vi "Status_Call.vi"(8 "error in (no error)":errorcluster, 9 "connection":T3={"host"="", "channel"=2, "cert path"=path "/home/lvuser/cansub_root_cert.crt"}, 10 "open in":bool, 11 "status client in":T2) -> (0 "error out":errorcluster, 1 "device status":T1, 2 "open out":bool, 3 "status client out":T2)   [LabVIEW 2021, in "CANsub_API.lvlib"]
doc: "Reads the device status with an HTTPS client that stays open between calls. Opens the client on the first call (about 80 ms for the TLS handshake). A later call takes about 1 ms. After an error, the client is closed, and the next call opens a new one."
uses:
  CANsub_API.lvlib
  common/CANsub_Common.lvlib
  <vilib>/httpClient/ClientHandle.ctl
  <vilib>/httpClient/LabVIEWHTTPClient.lvlib
  common/Typedefs/CANsub_connection.ctl
  common/Typedefs/CANsub_Device_Status.ctl
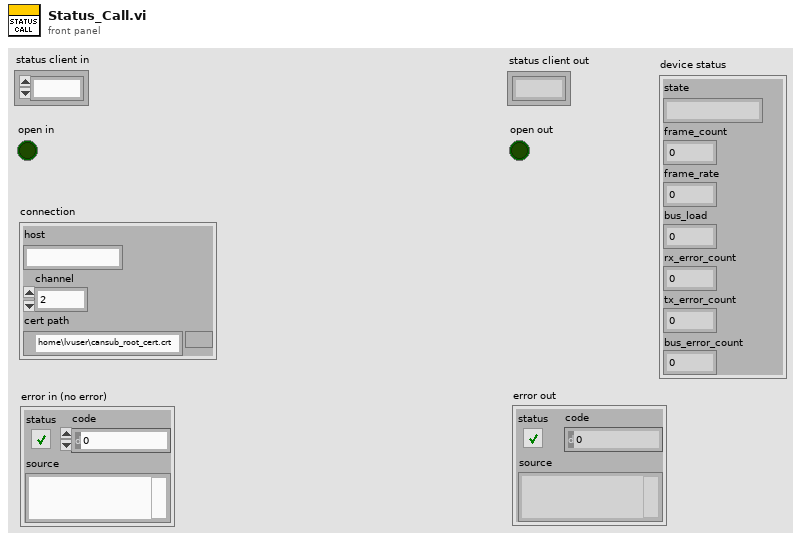
[diagram p1: front panel]
types:
  T1 = typedef "CANsub_Common.lvlib/CANsub_Device_Status.ctl" = cluster{"state":string, "frame_count":u32, "frame_rate":dbl, "bus_load":dbl, "rx_error_count":u32, "tx_error_count":u32, "bus_error_count":u32}
  T2 = typedef "LabVIEWHTTPClient.lvlib/ClientHandle.ctl" = refnum<k1>
  T3 = typedef "CANsub_Common.lvlib/CANsub_connection.ctl" = cluster{"host":string, "channel":u8, "cert path":path}
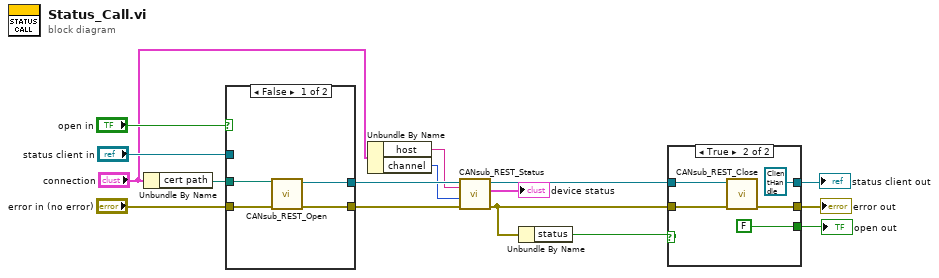
[diagram p0: block diagram]
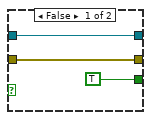
[diagram p3: hidden frame]
diagram:
  n1 = Unbundle By Name("connection") -> ("cert path"=w13:path)
  n2 = case shown="False" "open in" {
    tunnel: [w18 w22] -> w12
    tunnel: "status client in" -> [_ w22]
    tunnel: [w17 w21] -> w10
    tunnel: "error in (no error)" -> [w19 w21]
    tunnel: w13 -> [w20 _]
    frame False {
      n3 = call "CANsub_REST_Open.vi"("error in (no error)"=w19, "cert path"=w20) -> ("error out"=w17:errorcluster, "client handle"=w18:T2)  [unwired: 8 in]
    }
    frame True {
    }
  }
  n4 = Unbundle By Name("connection") -> ("host"=w3:string, "channel"=w2:u8)
  n5 = call "CANsub_REST_Status.vi"("error in (no error)"=w10, "channel"=w2, "host"=w3, "client handle"=w12) -> ("error out"=w6:errorcluster, "device status"=→"device status":T1, "client handle out"=w5:T2)  [unwired: 5 in]
  n6 = Unbundle By Name(w6) -> ("status"=w9:bool)
  n7 = case shown="True" w9 {
    tunnel: [TRUE FALSE] -> w8
    tunnel: [w24 w27] -> w7
    tunnel: w6 -> [w24 w28]
    tunnel: w5 -> [w23 w29]
    tunnel: [w23 T2 refnum ("client handle out")] -> w1
    frame False {
    }
    frame True {
      n8 = call "CANsub_REST_Close.vi"("error in (no error)"=w28, "client handle"=w29) -> ("error out"=w27:errorcluster)  [unwired: 9 in]
    }
  }
  "status client out" <- w1
  "open out" <- w8
  "error out" <- w7
